vi "KELLER.vi"() -> ()   [LabVIEW 2022 SP3]
uses:
  Enum/Enum k1.ctl
  <vilib>/Instr/_visa.llb/VISA Flush IO Buffer Mask.ctl
  Variables globales/Variable glob generale.vi
  Variables globales/Variable glob Keller.vi
panel:
  out "Adresses des Keller":u8[](array[numeric])=[10]
  out "Valeurs KELLER":string[](array[string])
  out "Port COM KELLER":refnum<visa-resource-name>="COM11"
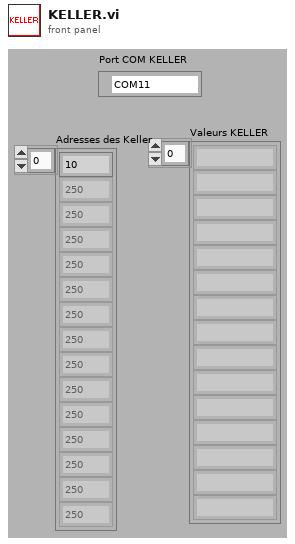
[diagram p1: front panel]
types:
  T1 = typedef "Enum k1.ctl" = enum16{"sélection", "init COM", "lecture"}
  T2 = typedef "VISA Flush IO Buffer Mask.ctl" = u16
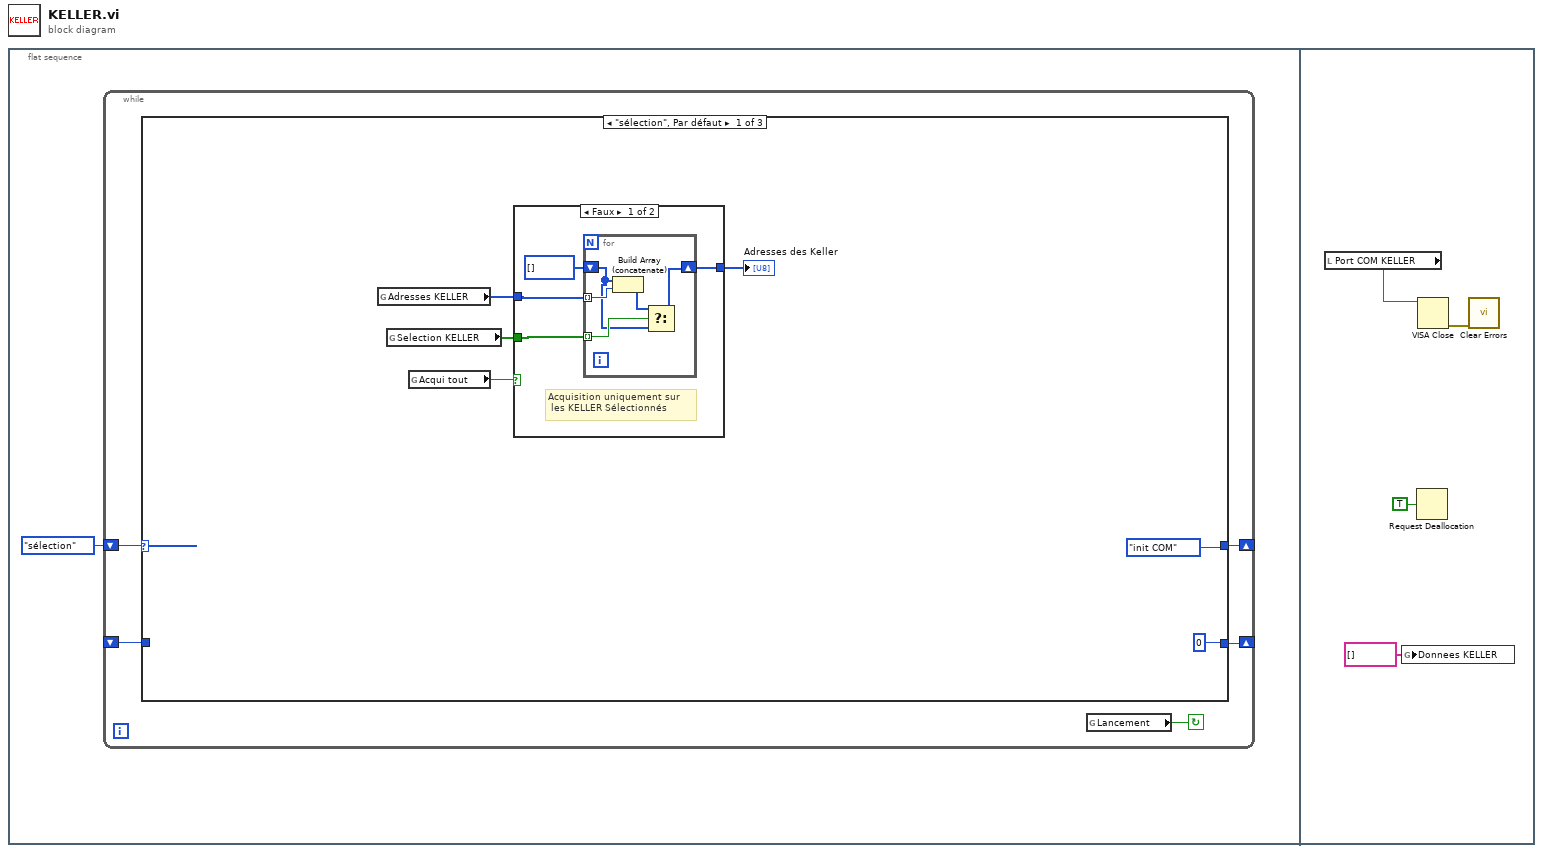
[diagram p0: block diagram]
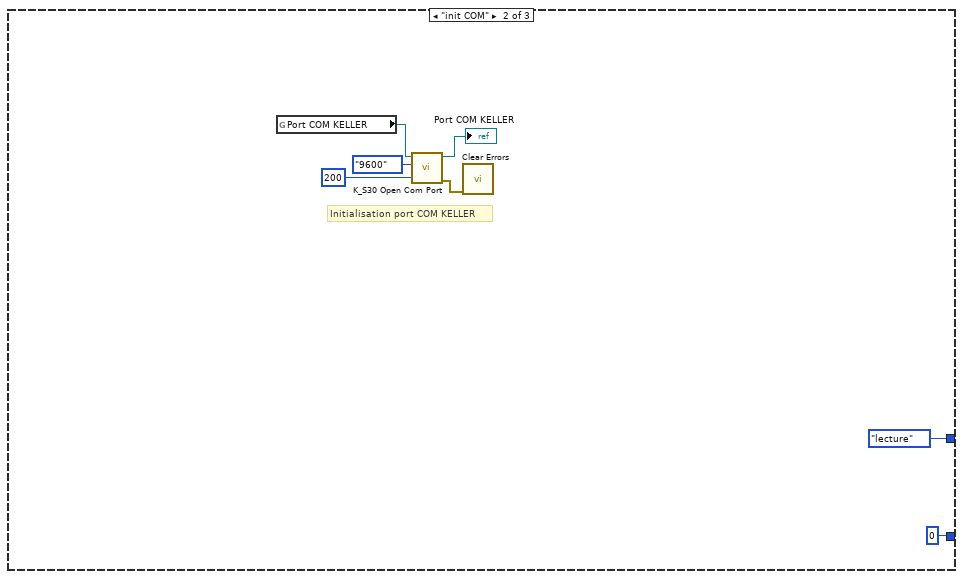
[diagram p3: hidden frame]
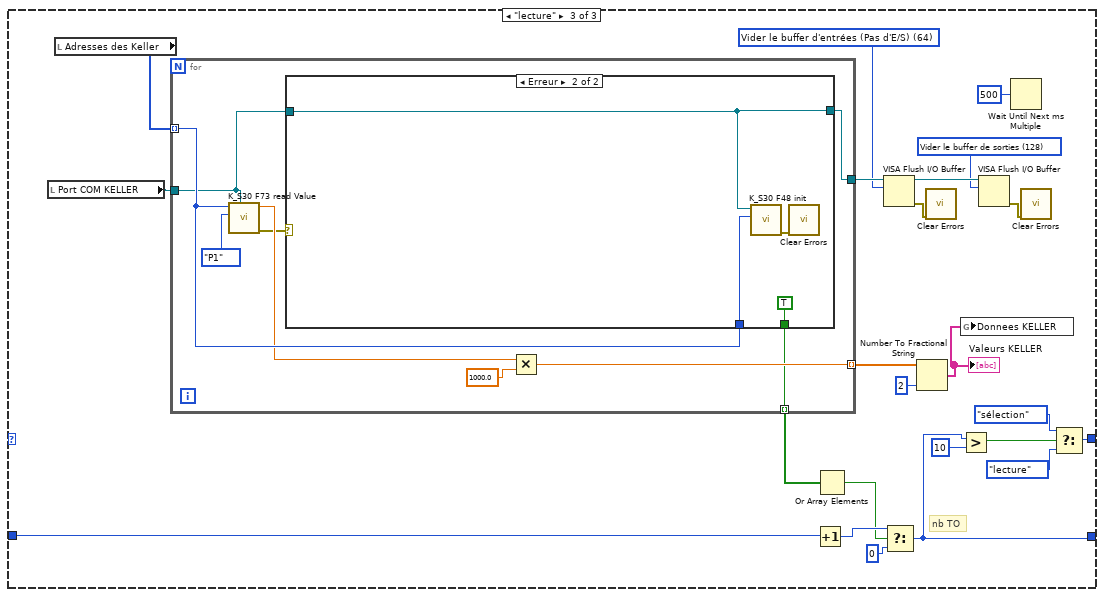
[diagram p4: hidden frame]
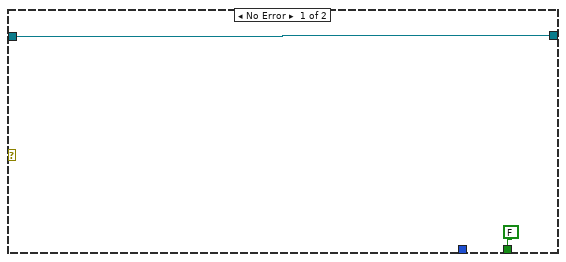
[diagram p5: hidden frame]
diagram:
  n1 = flat-sequence {
    frame #0 {
      n2 = while {
        shift-right: [w4] -> _
        shift-left: Enum_k1."sélection" ("Énum") -> [w5]
        shift-right: [w3] -> _
        shift-left: _ -> [w2]
        stop <- w6 continue-if-true
        n3 = case shown="\"sélection\", Par défaut" w5 {
          tunnel: [Enum_k1."init COM" ("Énum") Enum_k1."lecture" ("Énum") w35] -> w4
          tunnel: [0 0 w33] -> w3
          tunnel: w2 -> [_ _ w32]
          frame "sélection", Default {
            n4 = global read "Variable glob Keller.vi" "Adresses KELLER"() -> (w9:i16[])
            n5 = global read "Variable glob Keller.vi" "Selection KELLER"() -> (w10:bool[])
            n6 = global read "Variable glob generale.vi" "Acqui tout"() -> (w11:bool)
            n7 = case shown="Faux" w11 {
              tunnel: w9 -> [w16 w22]
              tunnel: w10 -> [w15 _]
              tunnel: [w13 w22] -> w12
              frame False {
                # "Acquisition uniquement sur\n les KELLER Sélectionnés"
                n8 = for {
                  tunnel: w16 -> [w20] mode=indexing
                  tunnel: w15 -> [w21] mode=indexing
                  shift-right: [w18] -> w13
                  shift-left: i8[] [] -> [w17]
                  n9 = Build Array (concatenate)(w17, w20) -> (w19:i16[])
                  n10 = Select(t=w19, s=w21, f=w17) -> (s? t:f=w18:i16[])
                }
              }
              frame True {
                # "Acquisition sur l'ensemble des\n KELLER configurés"
              }
            }
            "Adresses des Keller" <- w12
          }
          frame "init COM" {
            # "Initialisation port COM KELLER"
            n11 = global read "Variable glob Keller.vi" "Port COM KELLER"() -> (w26:refnum<visa-resource-name>)
            n12 = call "K_S30 Open Com Port.vi"("timeout"=u32 200, "Baudrate"=enum16{"9600", "115200"}."9600", "VISA resource name"=w26) -> ("error out"=w29:errorcluster, "VISA out"=→"Port COM KELLER":refnum<visa-resource-name>)  [unwired: 5 in]
            n13 = call <vilib>:"Clear Errors.vi"("error in (no error)"=w29) -> ()  [unwired: 5 in, 2 out]
          }
          frame "lecture" {
            w43 = T2 128 items=["Vider le buffer d'entrées"=16, "Écrire le buffer de sorties sur le périphérique"=32, "Vider le buffer d'entrées (Pas d'E/S)"=64, "Vider le buffer de sorties"=128] ("Mask")
            w46 = T2 64 items=["Vider le buffer d'entrées"=16, "Écrire le buffer de sorties sur le périphérique"=32, "Vider le buffer d'entrées (Pas d'E/S)"=64, "Vider le buffer de sorties"=128] ("Mask")
            # "nb TO"
            n14 = local read "Port COM KELLER"() -> (w41:refnum<visa-resource-name>)
            n15 = local read "Adresses des Keller"() -> (w42:u8[])
            n16 = for {
              tunnel: w41 -> [w54]
              tunnel: [w60] -> w51 mode=indexing
              tunnel: w42 -> [w58] mode=indexing
              tunnel: [w59] -> w48
              tunnel: [w53] -> w31 mode=indexing
              n17 = call "K_S30 F73 read Value.vi"("VISA resource"=w54, "Channel"=enum16{"CH0", "P1", "P2", "T", "TOB1", "TOB2"}."P1", "Address"=w58) -> ("error out"=w55:errorcluster, "Value"=w56:sgl)  [unwired: 6 in, 1 out]
              n18 = case shown="Erreur" w55 {
                tunnel: w54 -> [w63 w67]
                tunnel: [w63 w67] -> w59
                tunnel: w58 -> [_ w66]
                tunnel: [FALSE TRUE] -> w53
                frame No Error {
                }
                frame Error {
                  n19 = call "K_S30 F48 init.vi"("Address"=w66, "VISA resource"=w67) -> ("error out"=w65:errorcluster)  [unwired: 7 in, 2 out]
                  n20 = call <vilib>:"Clear Errors.vi"("error in (no error)"=w65) -> ()  [unwired: 5 in, 2 out]
                }
              }
              n21 = Multiply(x=w56, y=sgl 1000.0) -> (x*y=w60:sgl)
            }
            n22 = Increment(x=w32) -> (x+1=w40:i32)
            n23 = Or Array Elements(Boolean array=w31) -> (logical OR=w30:bool)
            n24 = VISA Flush I/O Buffer(VISA resource name=w48, mask (16)=w46) -> (VISA resource name out=w44:refnum<visa-resource-name>, error out=w47:errorcluster)  [unwired: 1 in]
            n25 = Select(t=w40, s=w30, f=0 ("cas faux")) -> (s? t:f=w33:i32)
            n26 = Number To Fractional String(number=w51, precision (6)=i16 2 ("précision (6)")) -> (F-format string=w49:string[])  [unwired: 2 in]
            "Valeurs KELLER" <- w49
            n27 = call <vilib>:"Clear Errors.vi"("error in (no error)"=w47) -> ()  [unwired: 5 in, 2 out]
            n28 = global write "Variable glob Keller.vi" "Donnees KELLER"(w49) -> ()
            n29 = Greater?(x=w33, y=10) -> (0:w34:bool)
            n30 = VISA Flush I/O Buffer(VISA resource name=w44, mask (16)=w43) -> (error out=w45:errorcluster)  [unwired: 1 in, 1 out]
            n31 = Wait Until Next ms Multiple(millisecond multiple=u32 500 ("n millisecondes")) -> ()  [unwired: 1 out]
            n32 = call <vilib>:"Clear Errors.vi"("error in (no error)"=w45) -> ()  [unwired: 5 in, 2 out]
            n33 = Select(t=Enum_k1."sélection" ("Énum"), s=w34, f=Enum_k1."lecture" ("Énum")) -> (s? t:f=w35:T1)
          }
        }
        n34 = global read "Variable glob generale.vi" "Lancement"() -> (w6:bool)
      }
    }
    frame #1 {
      n35 = local read "Port COM KELLER"() -> (w68:refnum<visa-resource-name>)
      n36 = global write "Variable glob Keller.vi" "Donnees KELLER"(string[] [] ("Données KELLER")) -> ()
      n37 = Request Deallocation(TRUE ("flag")) -> ()
      n38 = VISA Close(VISA resource name=w68) -> (error out=w70:errorcluster)  [unwired: 1 in]
      n39 = call <vilib>:"Clear Errors.vi"("error in (no error)"=w70) -> ()  [unwired: 5 in, 2 out]
    }
  }
